vi "lvmcp_subvipath.vi"() -> ()   [LabVIEW 2015]
panel:
  out "error out":errorcluster
  out "path":path
  in  "reference":refnum<vi>
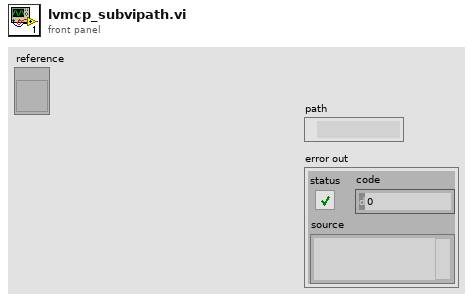
[diagram p1: front panel]
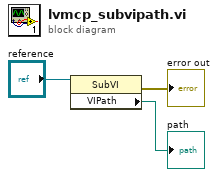
[diagram p0: block diagram]
diagram:
  n1 = property class="SubVI"(reference="reference") -> (error out=→"error out":errorcluster, "VIPath"=→"path":path)  [unwired: 1 in, 1 out]
